vi "Is a JKI State Machine.vi"(8 "error in (no error)":errorcluster, 11 "JKI SM in":refnum<class "JKI SM.lvclass">) -> (0 "error out":errorcluster, 2 "Is a JKI State Machine":bool, 3 "JKI SM out":refnum<class "JKI SM.lvclass">)   [LabVIEW 2020, in "JKI State Machine API.lvlib" / "JKI SM.lvclass"]
uses:
  JKI SM.lvclass
  JKI SM.lvclass/JKI SM.ctl
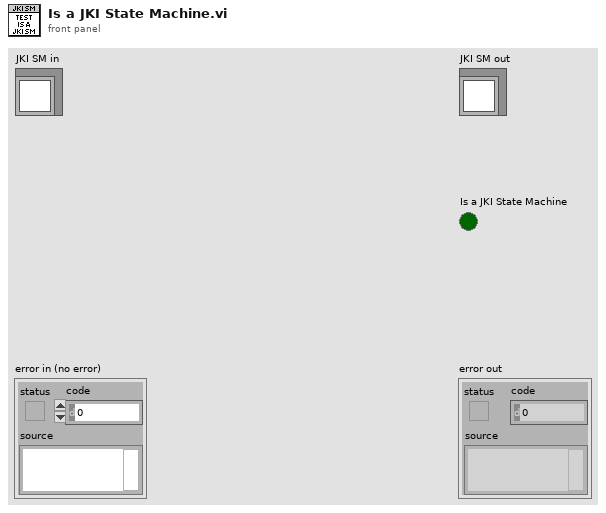
[diagram p1: front panel]
types:
  T1 = typedef "JKI State Machine API.lvlib/JKI SM.lvclass/Part References -- Cluster.ctl" = cluster{"While Loop":refnum<vi>, "Case Structure":refnum<vi>, "Event Structure":refnum<vi>, "Parse State Queue":refnum<vi>, "VI":refnum<vi>}
  T2 = cluster{"While Loop":bool, "Case Structure":bool, "Event Structure":bool, "Parse State Queue":bool, "VI":bool}
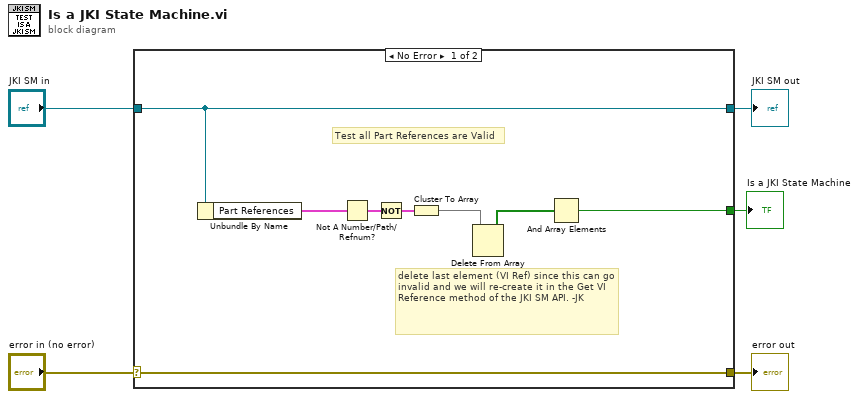
[diagram p0: block diagram]
diagram:
  n1 = case shown="No Error" "error in (no error)" {
    selector: "error in (no error)" -> [w13 w15]
    tunnel: [w13 w15] -> w4
    tunnel: [w12 w14] -> w2
    tunnel: "JKI SM in" -> [w12 w14]
    tunnel: [w9 _] -> w1
    frame No Error {
      # "delete last element (VI Ref) since this can go invalid and we will re-create it in the Get VI Reference method of the JKI SM API. -JK"
      # "Test all Part References are Valid"
      n2 = Unbundle By Name(w12) -> ("Part References"=w11:T1)
      n3 = Not A Number/Path/Refnum?(number/path/refnum=w11) -> (NaN/Path/Refnum?=w10:T2)
      n4 = Not(x=w10) -> (.not. x?=w8:T2)
      n5 = Cluster To Array(cluster=w8) -> (array=w7:bool[])
      n6 = Delete From Array(array=w7) -> (array with subset deleted=w6:bool[])  [unwired: 2 in, 1 out]
      n7 = And Array Elements(Boolean array=w6) -> (logical AND=w9:bool)
    }
    frame Error {
    }
  }
  "error out" <- w4
  "JKI SM out" <- w2
  "Is a JKI State Machine" <- w1
